vi "Open SequenceFile.vi"(7 "File Load Options":T1={"Use Search Dirs? (T)"=TRUE, "Conflict as Error? (T)"=TRUE, "Check Station Model? (F)"=FALSE, "Preload Modules? (T)"=TRUE, "Skip Load Callback? (F)"=FALSE, "Reload if Loaded? (F)"=FALSE}, 8 "error in (no error)":errorcluster, 9 "Current Seq File (None)":refnum<class "SequenceFile.lvclass">, 10 "File Path":path, 11 "Engine in":refnum<class "Engine.lvclass">) -> (0 "error out":errorcluster, 2 "SequenceFile":refnum<class "SequenceFile.lvclass">, 3 "Engine out":refnum<class "Engine.lvclass">)   [LabVIEW 2020, in "TSnax.lvlib" / "Engine.lvclass"]
uses:
  Engine.lvclass
  File Load Options.ctl
  SequenceFile/SequenceFile.lvclass
  SequenceFile Response.ctl
  Open SequenceFile Request.ctl
  Engine.lvclass/Engine.ctl
  d3fa0aa8-04a0-4514-abab-cbc7b376086a.vi
  TSnax.lvlib
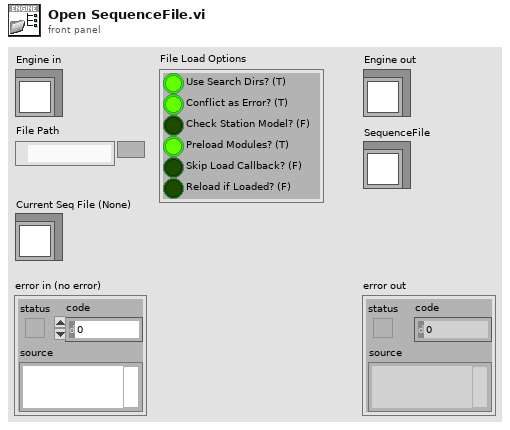
[diagram p1: front panel]
types:
  T1 = typedef "TSnax.lvlib/File Load Options.ctl" = cluster{"Use Search Dirs? (T)":bool, "Conflict as Error? (T)":bool, "Check Station Model? (F)":bool, "Preload Modules? (T)":bool, "Skip Load Callback? (F)":bool, "Reload if Loaded? (F)":bool}
  T2 = typedef "TSnax.lvlib/Engine.lvclass/Open SequenceFile Request.ctl" = cluster{"File Path":path, "File Load Options":T1, "Current SeqFile":refnum<class "SequenceFile.lvclass">, "Notifier":refnum<notifier>}
  T3 = typedef "TSnax.lvlib/Engine.lvclass/SequenceFile Response.ctl" = cluster{"SequenceFile":refnum<class "SequenceFile.lvclass">, "Error":errorcluster}
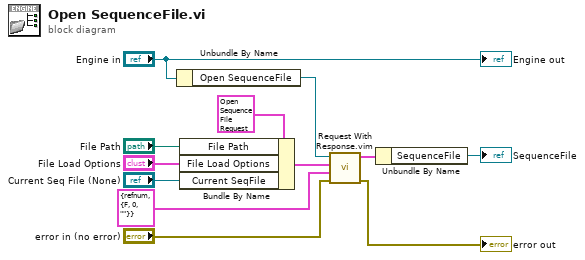
[diagram p0: block diagram]
diagram:
  n1 = Unbundle By Name("Engine in") -> ("Open SequenceFile"=w6:refnum<user-event>)
  n2 = Bundle By Name(cluster=T2 {"File Path"=path "", "File Load Options"={"Use Search Dirs? (T)"=TRUE, "Conflict as Error? (T)"=TRUE, "Check Station Model? (F)"=FALSE, "Preload Modules? (T)"=TRUE, "Skip Load Callback? (F)"=FALSE, "Reload if Loaded? (F)"=FALSE}, "Current SeqFile"=refnum, "Notifier"=refnum} ("event data"), "File Path"="File Path", "File Load Options"="File Load Options", "Current SeqFile"="Current Seq File (None)") -> (w7:T2)
  n3 = call "Request With Response.vim"("error in (no error)"="error in (no error)", "Response Default (Error Only)"=T3 {"SequenceFile"=refnum, "Error"={"status"=FALSE, "code"=0, "source"=""}} ("Open SequenceFile Response"), "Request Data"=w7, "Event"=w6) -> ("error out"=→"error out":errorcluster, "Response"=w2:T3)  [unwired: 6 in]
  n4 = Unbundle By Name(w2) -> ("SequenceFile"=→"SequenceFile":refnum<class "SequenceFile.lvclass">)
  "Engine out" <- "Engine in"
